vi "To XML.vi"(8 "error in (no error)":errorcluster, 9 "Parent":refnum<k20>, 10 "Document":refnum<k20>, 11 "Package in":refnum<class "Package.lvclass">) -> (0 "error out":errorcluster)   [LabVIEW 2017, in "Cobertura.lvlib" / "Package.lvclass"]
uses:
  Package.lvclass
  Package.lvclass/Package.ctl
  <vilib>/xml/Close Reference(Node).vi
  Class/Class.lvclass
  <resource>/objmgr/DOMUserDefRef.rc
  <vilib>/xml/NI_XML.lvlib
  Cobertura.lvlib
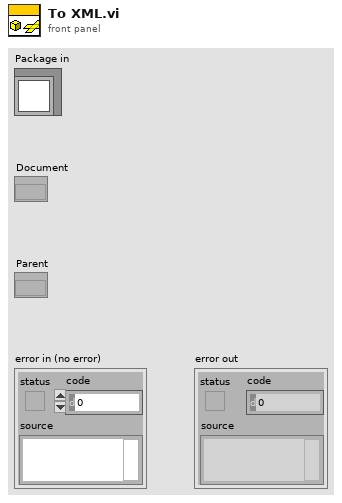
[diagram p1: front panel]
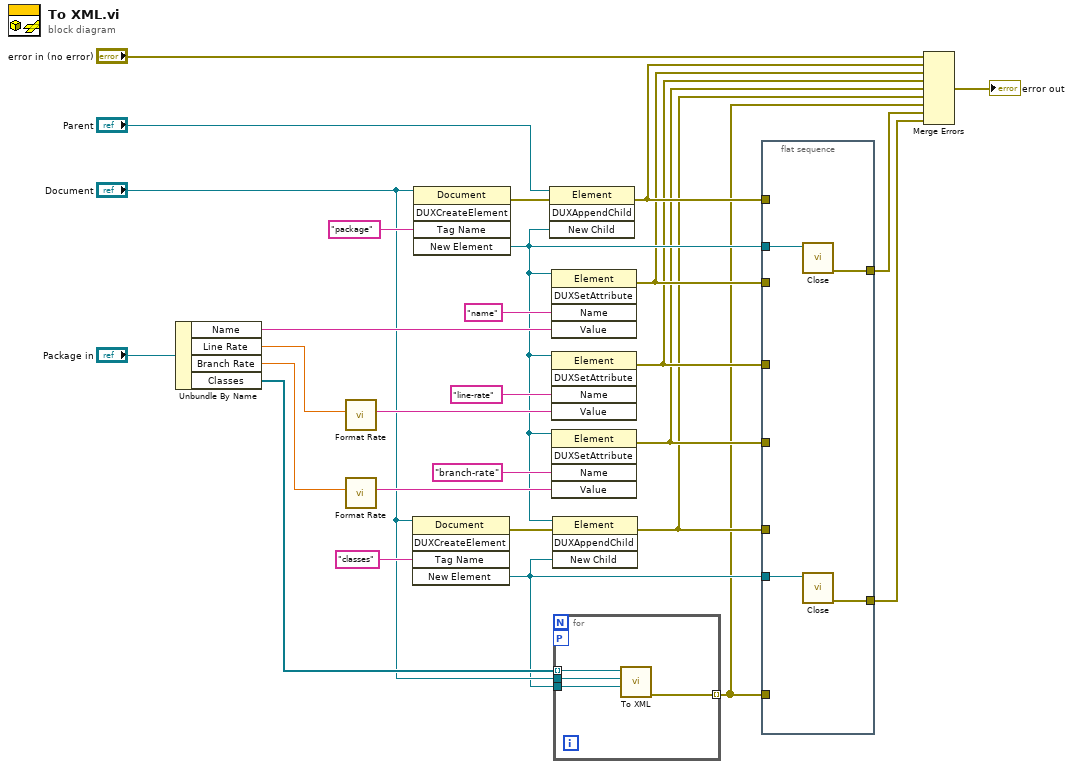
[diagram p0: block diagram]
diagram:
  n1 = Unbundle By Name("Package in") -> ("Name"=w22:string, "Line Rate"=w1:dbl, "Branch Rate"=w2:dbl, "Classes"=w20:refnum<class "Class.lvclass">[])
  n2 = call "Format Rate.vi"("Rate"=w1) -> ("String"=w26:string)  [unwired: 10 in]
  n3 = call "Format Rate.vi"("Rate"=w2) -> ("String"=w24:string)  [unwired: 10 in]
  n4 = invoke class="Document" method="DUXCreateElement"(reference="Document", "Tag Name"="classes") -> (error out=w16:errorcluster, "New Element"=w13:refnum<k20>)  [unwired: 3 in, 3 out]
  n5 = invoke class="Document" method="DUXCreateElement"(reference="Document", "Tag Name"="package") -> (error out=w15:errorcluster, "New Element"=w14:refnum<k20>)  [unwired: 3 in, 3 out]
  n6 = invoke class="Element" method="DUXAppendChild"(reference="Parent", error in=w15, "New Child"=w14) -> (error out=w12:errorcluster)  [unwired: 1 in, 3 out]
  n7 = invoke class="Element" method="DUXSetAttribute"(reference=w14, "Name"="name", "Value"=w22) -> (error out=w11:errorcluster)  [unwired: 2 in, 4 out]
  n8 = invoke class="Element" method="DUXSetAttribute"(reference=w14, "Name"="line-rate", "Value"=w26) -> (error out=w10:errorcluster)  [unwired: 2 in, 4 out]
  n9 = invoke class="Element" method="DUXSetAttribute"(reference=w14, "Name"="branch-rate", "Value"=w24) -> (error out=w9:errorcluster)  [unwired: 2 in, 4 out]
  n10 = invoke class="Element" method="DUXAppendChild"(reference=w14, error in=w16, "New Child"=w13) -> (error out=w8:errorcluster)  [unwired: 1 in, 3 out]
  n11 = for {
    tunnel: w20 -> [w32] mode=indexing
    tunnel: "Document" -> [w31]
    tunnel: w13 -> [w30]
    workers-P: _ -> [_]
    tunnel: [w29] -> w7 mode=indexing
    n12 = call-dynamic "To XML.vi"("Parent"=w30, "Document"=w31, "Class in"=w32) -> ("error out"=w29:errorcluster)  [unwired: 8 in]
  }
  n13 = flat-sequence {
    tunnel: w14 -> [w36]
    tunnel: w13 -> [w35]
    tunnel: w7 -> [_]
    tunnel: w8 -> [_]
    tunnel: w9 -> [_]
    tunnel: w10 -> [_]
    tunnel: w11 -> [_]
    tunnel: w12 -> [_]
    tunnel: [w34] -> w4
    tunnel: [w33] -> w3
    frame #0 {
      n14 = call-poly <vilib>:"Close.vi"("node"=w36) -> ("error out"=w34:errorcluster)  [unwired: 8 in]
      n15 = call-poly <vilib>:"Close.vi"("node"=w35) -> ("error out"=w33:errorcluster)  [unwired: 8 in]
    }
  }
  n16 = Merge Errors("error in (no error)", w12, w11, w10, w9, w8, w7, w4, w3) -> (→"error out":errorcluster)
